vi "Capture_Start.vi"(8 "error in (no error)":errorcluster={"status"=FALSE, "code"=0, "source"="\"\""}, 10 "parameter list":string, 11 "Run/step IDs":string) -> (0 "error out":errorcluster={"status"=FALSE, "code"=0, "source"="\"\""}, 2 "status ok":bool, 3 "CaptureSessionID":string)   [LabVIEW 2026]
doc: "INTENT: Open requested measurement session. LOGIC: Allocate bounded capture buffers, register selection and capture-window timing."
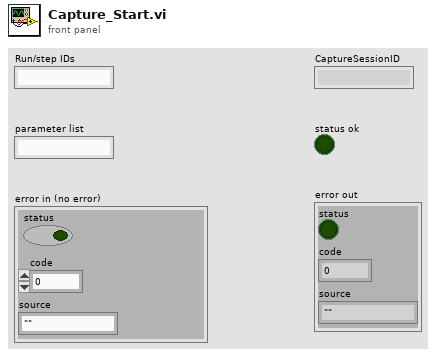
[diagram p1: front panel]
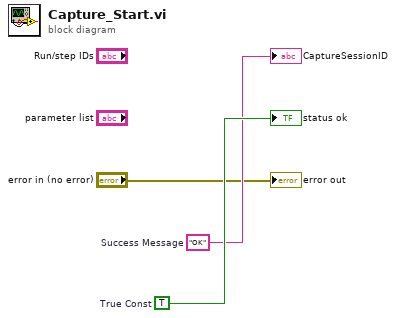
[diagram p0: block diagram]
diagram:
  w3 = TRUE  # True Const
  w2 = "OK"  # Success Message
  "CaptureSessionID" <- w2
  "status ok" <- w3
  "error out" <- "error in (no error)"
